vi "Missing PPLs on LV project.vi"(8 "error in (no error)":errorcluster, 11 "Path":path) -> (0 "error out":errorcluster, 3 "Pass":bool)   [LabVIEW 2021]
uses:
  <vilib>/addons/_JKI Toolkits/Caraya/classes/Assert/Assert False.vi
  <vilib>/addons/_JKI Toolkits/Caraya/classes/Assert/Assert.lvclass
  <vilib>/addons/_JKI Toolkits/Caraya/classes/Test/Test.lvclass
panel:
  out "Missing items from LabVIEW project":path[](array[path])
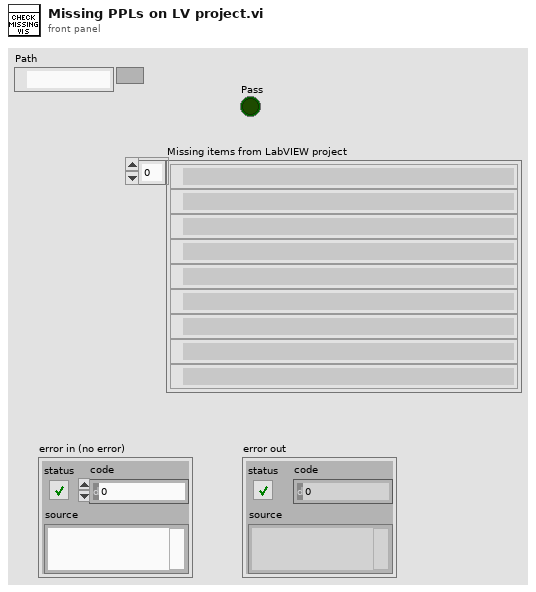
[diagram p1: front panel]
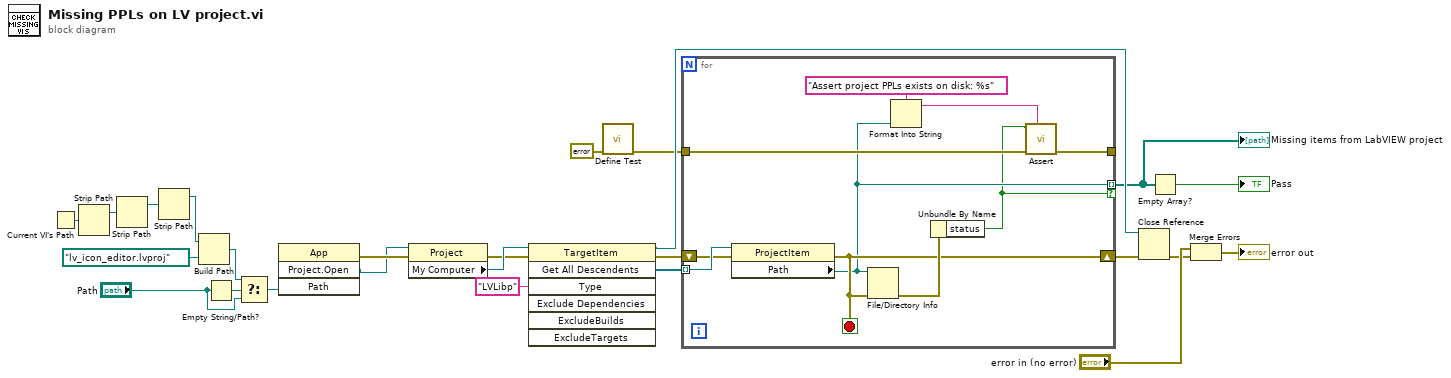
[diagram p0: block diagram]
diagram:
  n1 = Current VI's Path() -> (path=w6:path)
  n2 = Strip Path(path=w6) -> (stripped path=w5:path)  [unwired: 1 out]
  n3 = Strip Path(path=w5) -> (stripped path=w4:path)  [unwired: 1 out]
  n4 = Strip Path(path=w4) -> (stripped path=w3:path)  [unwired: 1 out]
  n5 = Build Path(base path=w3, name or relative path=path "lv_icon_editor.lvproj") -> (appended path=w7:path)
  n6 = Empty String/Path?(string/path="Path") -> (empty?=w8:bool)
  n7 = Select(t=w7, s=w8, f="Path") -> (s? t:f=w2:path)
  n8 = invoke class="App" method="Project.Open"("Path"=w2) -> (error out=w18:errorcluster, "Project:Open"=w17:refnum<vi>)  [unwired: 3 in, 2 out]
  n9 = property class="Project"(reference=w17, error in=w18) -> (error out=w22:errorcluster, "My Computer"=w25:refnum<vi>)  [unwired: 1 out]
  n10 = invoke class="TargetItem" method="Get All Descendents"(reference=w25, error in=w22, "Type"="LVLibp") -> (reference out=w19:refnum<vi>, error out=w21:errorcluster, "All Descendents"=w23:refnum<vi>[])  [unwired: 4 in, 4 out]
  n11 = call <vilib>:"Define Test.vi"("error in (no error)"=errorcluster {"status"=FALSE, "code"=0, "source"=""}) -> ("error out"=w11:errorcluster)  [unwired: 9 in, 1 out]
  n12 = for {
    tunnel: w23 -> [w35] mode=indexing
    shift-right: [w32] -> w20
    shift-left: w21 -> [w34]
    tunnel: [w27] -> w10 mode=indexing if=w26
    tunnel: w11 -> [w29]
    tunnel: [w28] -> _
    stop <- w32 stop-if-true
    n13 = property class="ProjectItem"(reference=w35, error in=w34) -> (error out=w32:errorcluster, "Path"=w27:path)  [unwired: 1 out]
    n14 = File/Directory Info(path=w27, error in=w32) -> (error out=w33:errorcluster)  [unwired: 6 out]
    n15 = Format Into String(format string="Assert project PPLs exists on disk: %s" ("Label"), w27) -> (resulting string=w31:string)  [unwired: 2 in, 1 out]
    n16 = Unbundle By Name(w33) -> ("status"=w26:bool)
    n17 = call-poly <vilib>:"Assert.vi"("Label"=w31, "error in (no error)"=w29, "False?"=w26) -> ("error out"=w28:errorcluster)  [unwired: 7 in, 1 out]
  }
  "Missing items from LabVIEW project" <- w10
  n18 = Close Reference(reference=w19, error in (no error)=w20) -> (error out=w14:errorcluster)
  n19 = Empty Array?(array=w10) -> (empty?=→"Pass":bool)
  n20 = Merge Errors("error in (no error)", w14) -> (→"error out":errorcluster)
